vi "RightClickMCLB.vi"(0 "VI Reference In":refnum<vi>, 5 "Control Ref In":refnum<vi>, 7 "Row":i32, 9 "Column":i32, 11 "Error In":errorcluster, 12 "Select Offset":i32) -> (4 "VI Reference Out":refnum<vi>, 6 "Control Ref Out":refnum<vi>, 15 "Error Out":errorcluster)   [LabVIEW 2019, in "Drona.lvlib"]
doc: "This VI performs right click function on MCLB in given row and column"
uses:
  Drona.lvlib
  Controls/ClickFunction.ctl
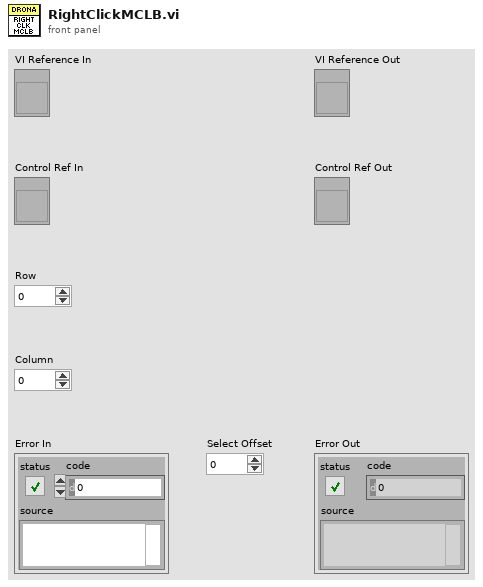
[diagram p1: front panel]
types:
  T1 = typedef "Drona.lvlib/ClickFunction.ctl" = enum16{"RightClickUp", "RightClickDown", "LeftClickUp", "LeftClickDown"}
  T2 = typedef "LVPositionTypeDef.ctl" = cluster{"Left":i32, "Top":i32}
  T3 = typedef "LVBoundsTypeDef.ctl" = cluster{"Width":u32, "Height":u32}
  T4 = typedef "LVRectTypeDef.ctl" = cluster{"Left":i16, "Top":i16, "Right":i16, "Bottom":i16}
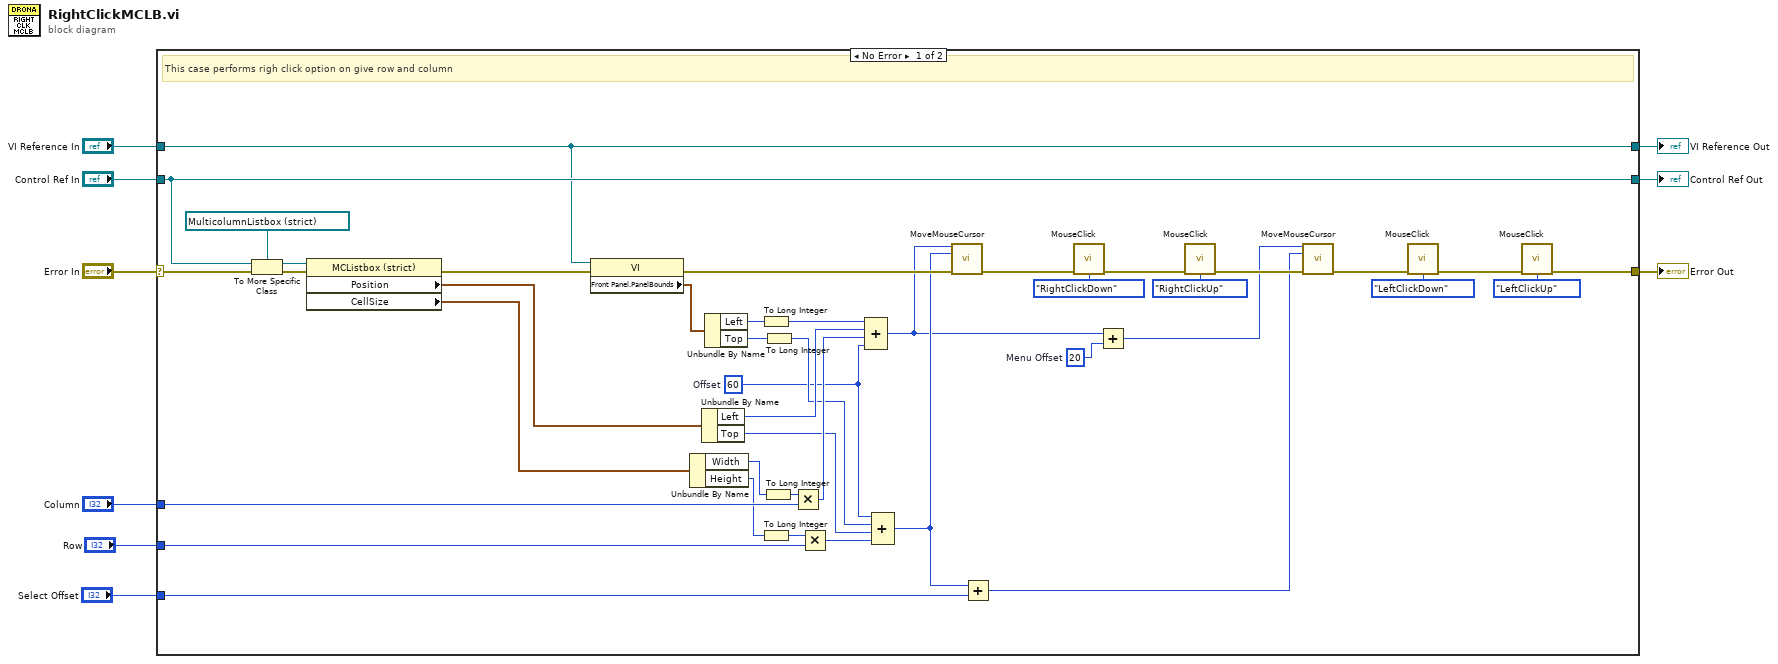
[diagram p0: block diagram]
diagram:
  n1 = case shown="No Error" "Error In" {
    selector: "Error In" -> [w51 w54]
    tunnel: "VI Reference In" -> [w34 w52]
    tunnel: "Control Ref In" -> [w36 w53]
    tunnel: "Row" -> [w17 _]
    tunnel: "Column" -> [w25 _]
    tunnel: "Select Offset" -> [w33 _]
    tunnel: [w37 w54] -> w3
    tunnel: [w34 w52] -> w1
    tunnel: [w36 w53] -> w2
    frame No Error {
      w10 = 20  # Menu Offset
      w15 = 60  # Offset
      # "This case performs righ click option on give row and column"
      n2 = To More Specific Class(target class=refnum<vi> refnum ("Multicolumn Listbox"), reference=w36, error in=w51) -> (specific class reference=w48:refnum<vi>, error out=w50:errorcluster)
      n3 = property class="MCListbox (strict)"(reference=w48, error in=w50) -> (error out=w47:errorcluster, "Position"=w29:T2, "CellSize"=w28:T3)  [unwired: 1 out]
      n4 = property class="VI"(reference=w34, error in=w47) -> (error out=w35:errorcluster, "Front Panel.PanelBounds"=w32:T4)  [unwired: 1 out]
      n5 = Unbundle By Name(w28) -> ("Width"=w26:u32, "Height"=w18:u32)
      n6 = Unbundle By Name(w29) -> ("Left"=w27:i32, "Top"=w22:i32)
      n7 = Unbundle By Name(w32) -> ("Left"=w31:i16, "Top"=w21:i16)
      n8 = To Long Integer(number=w31) -> (32bit integer=w30:i32)
      n9 = To Long Integer(number=w18) -> (32bit integer=w19:i32)
      n10 = To Long Integer(number=w26) -> (32bit integer=w24:i32)
      n11 = To Long Integer(number=w21) -> (32bit integer=w20:i32)
      n12 = Multiply(x=w24, y=w25) -> (x*y=w23:i32)
      n13 = Multiply(x=w19, y=w17) -> (x*y=w16:i32)
      n14 = Compound Arithmetic op=ADD(w30, w27, w23, w15) -> (w12:i32)
      n15 = Compound Arithmetic op=ADD(w15, w20, w22, w16) -> (w14:i32)
      n16 = call "MoveMouseCursor.vi"("Left Position"=w12, "Right Position"=w14, "Error In"=w35) -> ("Error Out"=w46:errorcluster)  [unwired: 12 in]
      n17 = Add(x=w14, y=w33) -> (x+y=w13:i32)
      n18 = call "MouseClick.vi"("Error In"=w46, "ClickFunction"=ClickFunction."RightClickDown") -> ("Error Out"=w44:errorcluster)  [unwired: 13 in]
      n19 = Add(x=w12, y=w10) -> (x+y=w11:i32)
      n20 = call "MouseClick.vi"("Error In"=w44, "ClickFunction"=ClickFunction."RightClickUp") -> ("Error Out"=w42:errorcluster)  [unwired: 13 in]
      n21 = call "MoveMouseCursor.vi"("Left Position"=w11, "Right Position"=w13, "Error In"=w42) -> ("Error Out"=w41:errorcluster)  [unwired: 12 in]
      n22 = call "MouseClick.vi"("Error In"=w41, "ClickFunction"=ClickFunction."LeftClickDown") -> ("Error Out"=w39:errorcluster)  [unwired: 13 in]
      n23 = call "MouseClick.vi"("Error In"=w39, "ClickFunction"=ClickFunction."LeftClickUp") -> ("Error Out"=w37:errorcluster)  [unwired: 13 in]
    }
    frame Error {
      # "If error, this case pass that error message only"
    }
  }
  "Error Out" <- w3
  "Control Ref Out" <- w2
  "VI Reference Out" <- w1
